vi "velocity-rms-kurtosis-test.vi"(4 "Kurtosis Tolerance":dbl=0.05, 5 "Velocity Tolerance (%)":dbl=2.0, 6 "Number of Blocks":i32=8, 7 "Samples per Block":i32=12800, 8 "error in (no error)":errorcluster, 9 "Sample Rate (S/s)":dbl=51200.0, 10 "Amplitude (g pk)":dbl=1.0, 11 "Frequency (Hz)":dbl=159.15) -> (0 "error out":errorcluster, 1 "Expected Velocity RMS (mm/s)":dbl, 2 "Velocity RMS (mm/s)":dbl, 3 "PASS":bool)   [LabVIEW 2026, in "Unit-Test.lvlib"]
doc: "PURPOSE\nUnit test for the two channels added to PowerSpectrum.vi (Calculations.lvlib): Velocity RMS and Kurtosis. Checks the g->m/s2 scaling, the SVL Integration setup (single integration, mm, 10 Hz highpass) and the Build Array order.\n\nHOW IT WORKS\n1. Synthesises a continuous-phase sine (Amplitude g pk at Frequency Hz, fs = Sample Rate) and cuts it into blocks of Samples per Block, like FlexLogger feeds Process.vi.\n2. Calls PowerSpectrum.vi once per block from ONE call site, so the integration filter state carries over between blocks as in the plugin. Early blocks show the highpass start-up transient.\n3. Reads the LAST TWO waveforms of Array of Waveforms: second-to-last = Kurtosis (Kurt), last = Velocity RMS (VelRMS). Matches the Initialize.vi name lists: PBand, Crest, Peak, RMS, Max, Min, Max-Min, Skew, Kurt, VelRMS.\n4. Compares the final block with the theory.\n\nEXPECTED (pure sine)\nVelocity RMS [mm/s] = A x 9806.65 / (2 pi f) / sqrt(2). Default 1 g pk at 159.15 Hz = 6.94 mm/s.\nKurtosis = 1.5 (sine). Gaussian noise = 3. Impacts > 3.\n\nHOW TO USE\nRun with the defaults. PASS = both checks true.\n- Velocity 1000x low: the g->mm/s2 multiply is 9.80665 instead of 9806.65 (SVL Integration with length units = mm expects mm/s2 in).\n- Values swapped: Build Array order wrong.\n- Kurtosis about -1.5: the VI reports excess kurtosis.\nVelocity RMS per Block shows the filter settling. Parameter Count must be 10 (the number of names in Initialize.vi)."
uses:
  Unit-Test.lvlib
  src/Vibration-Core/Calculations.lvlib
panel:
  out "Parameter Count":i32
  out "Kurtosis per Block":dbl[](array[numeric])
  out "Velocity RMS per Block":dbl[](array[numeric])
  out "Kurtosis PASS":bool
  out "Kurtosis":dbl
  out "Velocity PASS":bool
  out "Velocity Error (%)":dbl
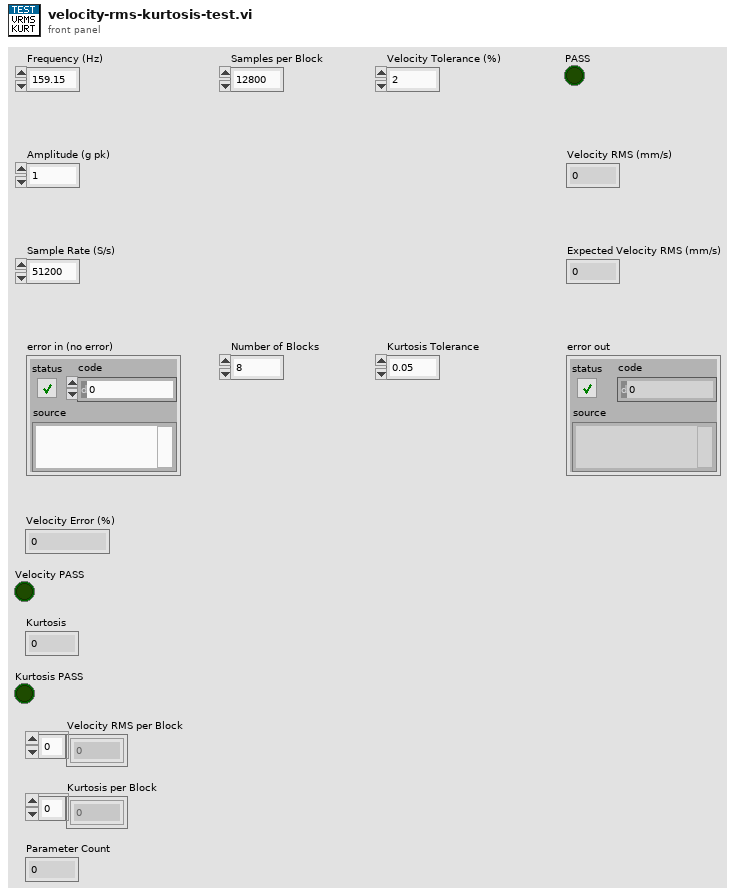
[diagram p1: front panel]
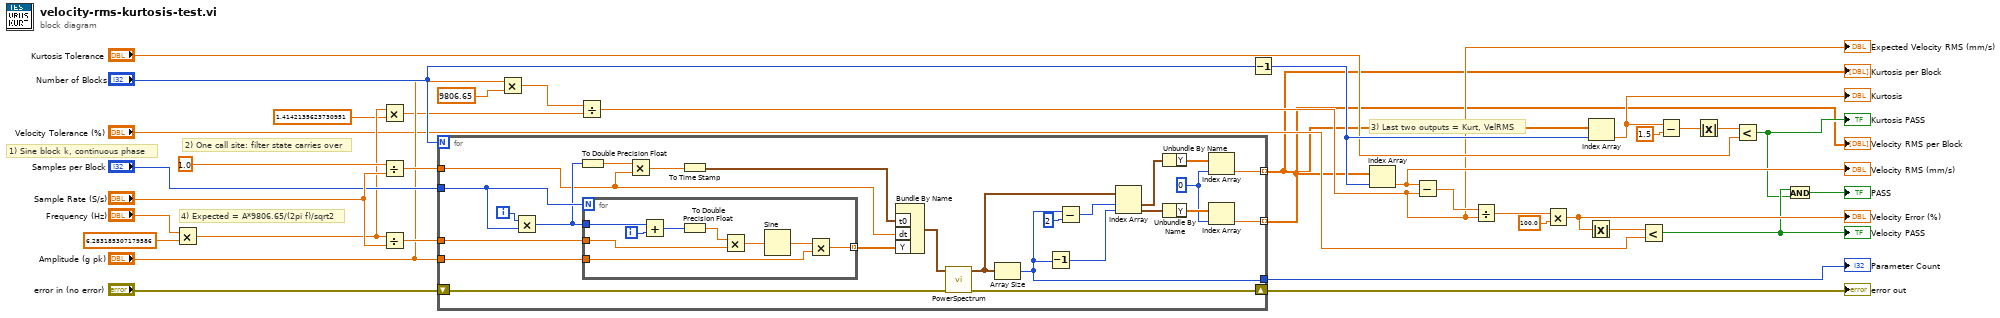
[diagram p0: block diagram]
diagram:
  # "4) Expected = A*9806.65/(2pi f)/sqrt2"
  # "3) Last two outputs = Kurt, VelRMS"
  # "2) One call site: filter state carries over"
  # "1) Sine block k, continuous phase"
  n1 = Multiply(x="Frequency (Hz)", y=6.283185307179586 ("2 pi")) -> (x*y=w24:dbl)
  n2 = Multiply(x=w24, y=1.4142135623730951 ("sqrt2")) -> (x*y=w21:dbl)
  n3 = Divide(x=1.0 ("one"), y="Sample Rate (S/s)") -> (x/y=w29:dbl)
  n4 = Divide(x=w24, y="Sample Rate (S/s)") -> (x/y=w30:dbl)
  n5 = for {
    N: "Number of Blocks" -> [_]
    shift-right: [w50] -> w1
    shift-left: "error in (no error)" -> [w51]
    tunnel: "Samples per Block" -> [w59]
    tunnel: w30 -> [w61]
    tunnel: "Amplitude (g pk)" -> [w60]
    tunnel: w29 -> [w54]
    tunnel: [w40] -> w4 mode=indexing
    tunnel: [w39] -> w3 mode=indexing
    tunnel: [w38] -> w2
    i -> [w37]
    w41 = 0 ("first")
    n6 = Multiply(x=w37, y=w59) -> (x*y=w58:i32)
    n7 = To Double Precision Float(number=w58) -> (double precision float=w57:dbl)
    n8 = for {
      N: w59 -> [_]
      tunnel: w58 -> [w70]
      tunnel: w61 -> [w67]
      tunnel: w60 -> [w64]
      tunnel: [w63] -> w53 mode=indexing
      i -> [w62]
      n9 = Add(x=w70, y=w62) -> (x+y=w69:i32)
      n10 = To Double Precision Float(number=w69) -> (double precision float=w68:dbl)
      n11 = Multiply(x=w68, y=w67) -> (x*y=w66:dbl)
      n12 = Sine(x=w66) -> (sin(x)=w65:dbl)
      n13 = Multiply(x=w65, y=w64) -> (x*y=w63:dbl)
    }
    n14 = Multiply(x=w57, y=w54) -> (x*y=w56:dbl)
    n15 = To Time Stamp(1:w56) -> (0:w55:timestamp)
    n16 = Bundle By Name("t0"=w55, "dt"=w54, "Y"=w53) -> (w52:waveform(dbl))  [unwired: 1 in]
    n17 = call "PowerSpectrum.vi"("error in (no error)"=w51, "Data In"=w52) -> ("error out"=w50:errorcluster, "Array of Waveforms"=w48:waveform(dbl)[])  [unwired: 7 in, 1 out]
    n18 = Array Size(array=w48) -> (size(s)=w38:i32)
    n19 = Decrement(x=w38) -> (x-1=w46:i32)
    n20 = Subtract(x=w38, y=2 ("two")) -> (x-y=w47:i32)
    n21 = Index Array(array=w48, index #1=w47, index #2=w46) -> (element #1=w45:waveform(dbl), element #2=w44:waveform(dbl))
    n22 = Unbundle By Name(w45) -> ("Y"=w43:dbl[])
    n23 = Unbundle By Name(w44) -> ("Y"=w42:dbl[])
    n24 = Index Array(array=w43, index=w41) -> (element=w39:dbl)
    n25 = Index Array(array=w42, index=w41) -> (element=w40:dbl)
  }
  "Velocity RMS per Block" <- w4
  "Kurtosis per Block" <- w3
  "Parameter Count" <- w2
  "error out" <- w1
  n26 = Multiply(x="Amplitude (g pk)", y=9806.65 ("g to mm/s2")) -> (x*y=w22:dbl)
  n27 = Divide(x=w22, y=w21) -> (x/y=w9:dbl)
  "Expected Velocity RMS (mm/s)" <- w9
  n28 = Decrement(x="Number of Blocks") -> (x-1=w27:i32)
  n29 = Index Array(array=w4, index=w27) -> (element=w10:dbl)
  "Velocity RMS (mm/s)" <- w10
  n30 = Subtract(x=w10, y=w9) -> (x-y=w20:dbl)
  n31 = Divide(x=w20, y=w9) -> (x/y=w19:dbl)
  n32 = Multiply(x=w19, y=100.0 ("percent")) -> (x*y=w8:dbl)
  "Velocity Error (%)" <- w8
  n33 = Absolute Value(x=w8) -> (abs(x)=w17:dbl)
  n34 = Index Array(array=w3, index=w27) -> (element=w6:dbl)
  "Kurtosis" <- w6
  n35 = Less?(x=w17, y="Velocity Tolerance (%)") -> (x < y?=w7:bool)
  "Velocity PASS" <- w7
  n36 = Subtract(x=w6, y=1.5 ("sine kurtosis")) -> (x-y=w14:dbl)
  n37 = Absolute Value(x=w14) -> (abs(x)=w13:dbl)
  n38 = Less?(x=w13, y="Kurtosis Tolerance") -> (x < y?=w5:bool)
  "Kurtosis PASS" <- w5
  n39 = And(x=w7, y=w5) -> (x .and. y?=→"PASS":bool)
